vi "flat sequence.vi"() -> ()   [LabVIEW 2016]
panel:
  out "String":string
  in  "Stop":bool
  out "Chart":dbl(graph)
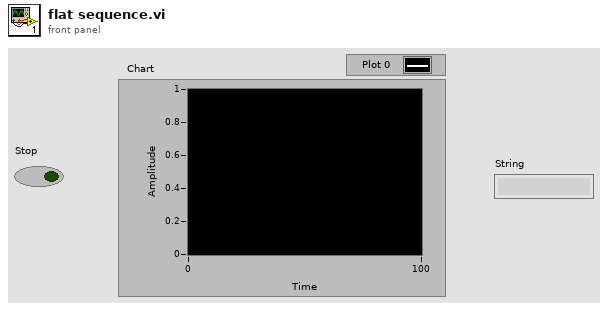
[diagram p1: front panel]
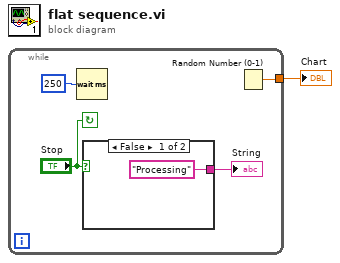
[diagram p0: block diagram]
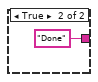
[diagram p2: hidden frame]
diagram:
  n1 = while {
    tunnel: [w4] -> w1
    stop <- "Stop" continue-if-true
    n2 = Wait (ms)(milliseconds to wait=u32 250) -> ()  [unwired: 1 out]
    n3 = case shown="False" "Stop" {
      tunnel: ["Processing" "Done"] -> w2
      frame False {
      }
      frame True {
      }
    }
    "String" <- w2
    n4 = Random Number (0-1)() -> (number: 0 to 1=w4:dbl)
  }
  "Chart" <- w1
